vi "FX_ReadFrame.vi"(10 "Words":u16, 11 "D":u16) -> (3 "Frame":string)   [LabVIEW 2018]
doc: "Use this template to build a VI to use as a subVI."
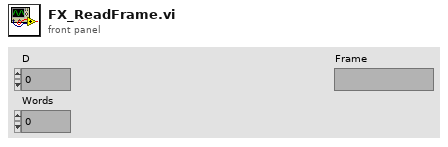
[diagram p1: front panel]
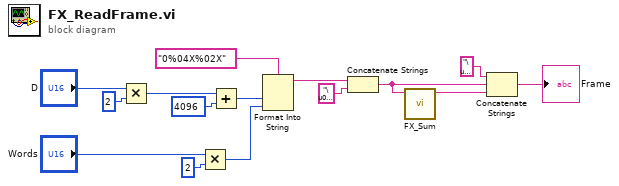
[diagram p0: block diagram]
diagram:
  n1 = Multiply(x="D", y=u16 2) -> (x*y=w13:u16)
  n2 = Multiply(x="Words", y=u16 2) -> (x*y=w7:u16)
  n3 = Add(x=w13, y=u16 4096) -> (x+y=w8:u16)
  n4 = Format Into String(format string="0%04X%02X", w8, w7) -> (resulting string=w6:string)  [unwired: 2 in, 1 out]
  n5 = Concatenate Strings(w6, "\u0003") -> (w4:string)
  n6 = call "FX_Sum.vi"("Body"=w4) -> ("SS"=w2:string)  [unwired: 10 in]
  n7 = Concatenate Strings("\u0002", w4, w2) -> (→"Frame":string)
